vi "WaitForMessageFromAddons.vi"(8 "error in (no error)":errorcluster, 9 "timeout ms":i32=200, 10 "Name":string="Diagnostic Unlock ECU Service", 11 "TCP Ref":refnum<k5>) -> (0 "error out":errorcluster)   [LabVIEW 2024, in "Diagnostic Unlock ECU Service.lvlib"]
uses:
  Diagnostic Unlock ECU Service.lvlib
  <vilib>/NI/STM/SubVIs/MetaDataElement.ctl
  <vilib>/NI/STM/TCP/TCP Read Options.ctl
  <vilib>/NI/NI VeriStand Addon Network Comm/Shared/_Types/Comm Message.ctl
  Service Shared/UnlockECU.SendSeedToWindowsAndWaitOnKeyCmd.ctl
  Service Shared/UnlockECU.SendSeedToWindowsAndWaitOnKeyResp.ctl
  <vilib>/NI/STM/TCP/TCP Write Options.ctl
  <vilib>/NI/STM/TCP/Write Meta Data (TCP Ref).vi
  <vilib>/NI/STM/TCP/Get Connection Reference (TCP).vi
  <vilib>/NI/STM/TCP/Write Meta Data (TCP Clst).vi
  <vilib>/NI/STM/TCP/Read Message (TCP).vi
  <vilib>/NI/STM/TCP/Write Message (TCP).vi
  <vilib>/NI/STM/NI STM.lvlib
  <vilib>/Utility/SystemLogging/NI_SystemLogging.lvlib
  Service Shared/Diagnostic Unlock ECU Service Shared.lvlib
  <vilib>/NI/NI VeriStand Addon Network Comm/Shared/NI VeriStand Addon Network Comm Shared.lvlib
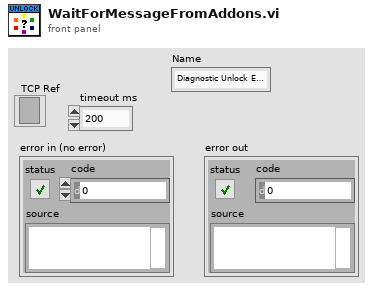
[diagram p1: front panel]
types:
  T1 = typedef "NI STM.lvlib/MetaDataElement.ctl" = string
  T2 = typedef "NI STM.lvlib/TCP Read Options.ctl" = cluster{"ignore timeout error":bool, "timeout ms (1000)":i32}
  T3 = typedef "NI VeriStand Addon Network Comm Shared.lvlib/Comm Message.ctl" = cluster{"Timeout":u32, "Resp?":bool, "data":string}
  T4 = typedef "NI STM.lvlib/TCP Write Options.ctl" = cluster{"ignore timeout error":bool, "timeout ms (1000)":i32}
  T5 = typedef "Diagnostic Unlock ECU Service Shared.lvlib/UnlockECU.SendSeedToWindowsAndWaitOnKeyResp.ctl" = cluster{"DLL Error":errorcluster, "Key Length":u32, "Key":u8[]}
  T6 = typedef "Diagnostic Unlock ECU Service Shared.lvlib/UnlockECU.SendSeedToWindowsAndWaitOnKeyCmd.ctl" = cluster{"Source DLL Path":path, "Security Level":u32, "Max Key Length":u32, "Seed":u8[], "ECU  Variant":i8, "Addon Name":string, "Optional Parameter":i8}
  T7 = typedef "NI STM.lvlib/TCP Connection Info.ctl" = cluster{"connection ID":refnum<k5>, "meta data":T1[]}
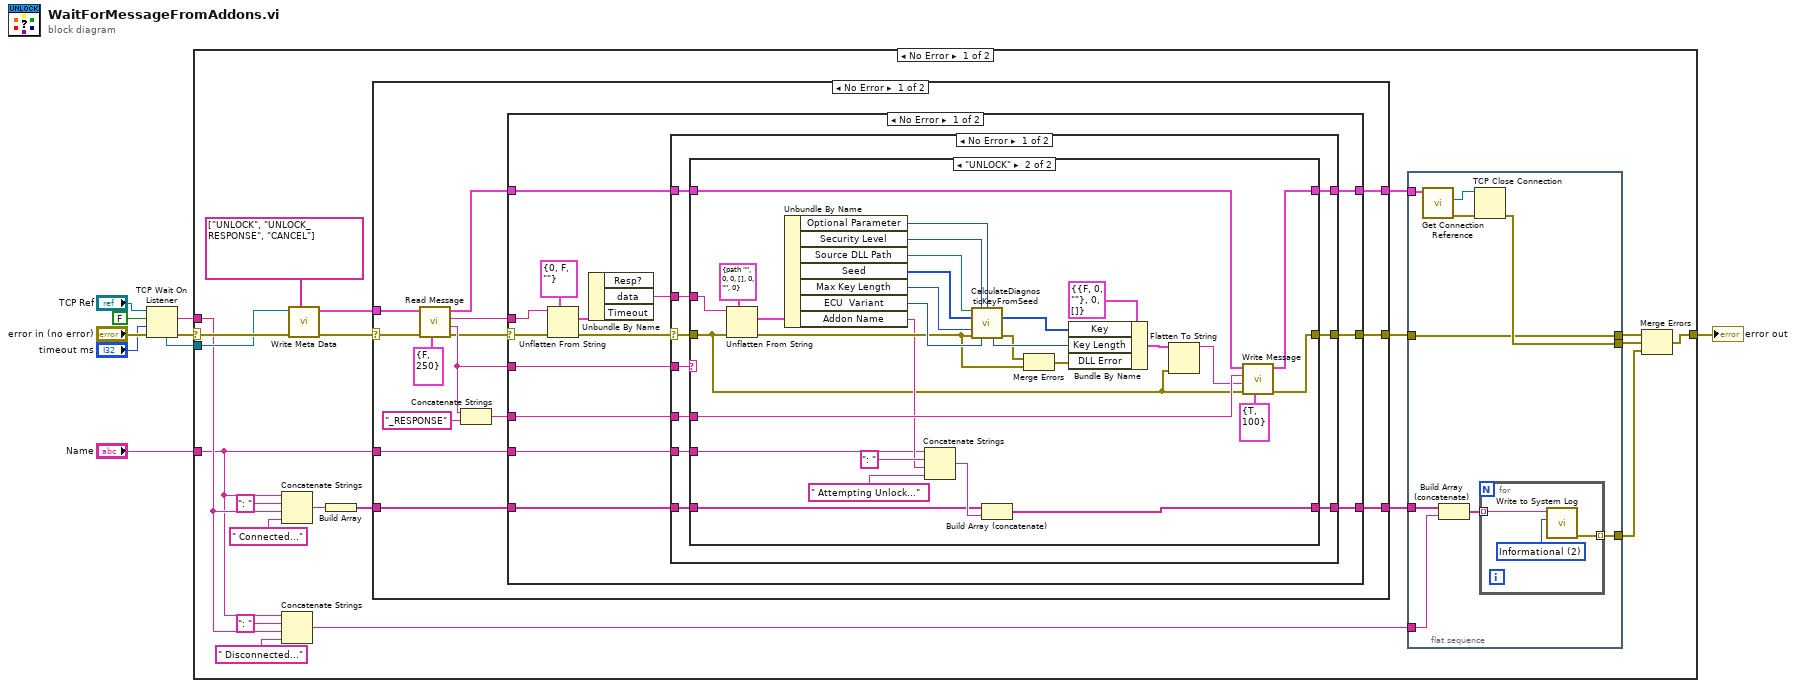
[diagram p0: block diagram]
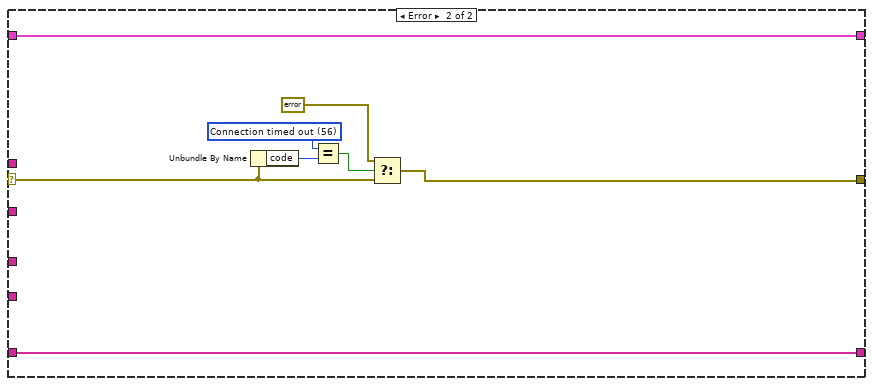
[diagram p4: hidden frame]
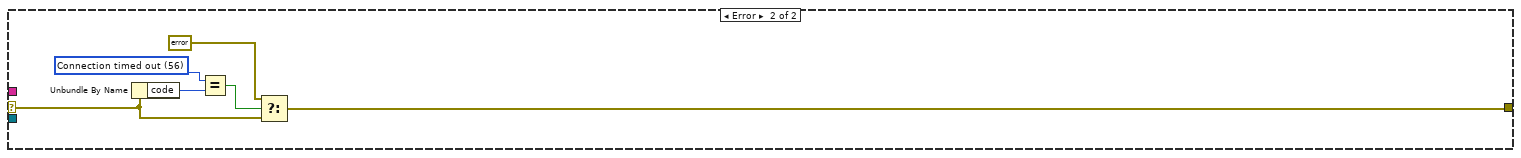
[diagram p6: hidden frame]
diagram:
  n1 = TCP Wait On Listener(8:"error in (no error)", 9:"timeout ms", 10:FALSE ("resolve remote address (T)"), 11:"TCP Ref") -> (0:w2:errorcluster, 2:w9:string, 4:w7:refnum<k5>)  [unwired: 2 out]
  n2 = case shown="No Error" w2 {
    selector: w2 -> [w30 w129]
    tunnel: [w24 w128] -> w1
    tunnel: w7 -> [w29 _]
    tunnel: w9 -> [w13 _]
    tunnel: "Name" -> [w12 _]
    frame No Error {
      n3 = Concatenate Strings(w12, ": " ("string"), w13, " Connected..." ("string")) -> (w19:string)
      n4 = Concatenate Strings(w12, ": " ("string"), w13, " Disconnected..." ("string")) -> (w11:string)
      n5 = call-poly <vilib>:"Write Meta Data.vi"("meta data"=T1[] ["UNLOCK", "UNLOCK_RESPONSE", "CANCEL"], "error in"=w30, "connection ID"=w29) -> ("error out"=w27:errorcluster, "connection info out"=w28:T7)  [unwired: 7 in]
      n6 = Build Array(w19) -> (w18:string[])
      n7 = case shown="No Error" w27 {
        selector: w27 -> [w46 w127]
        tunnel: [w48 w127] -> w22
        tunnel: w28 -> [w56 w126]
        tunnel: [w47 w126] -> w26
        tunnel: w12 -> [w45 _]
        tunnel: w18 -> [w44 w125]
        tunnel: [w43 w125] -> w17
        frame No Error {
          n8 = call-poly <vilib>:"Read Message.vi"("options"=T2 {"ignore timeout error"=FALSE, "timeout ms (1000)"=250}, "error in"=w46, "connection info in"=w56) -> ("error out"=w51:errorcluster, "name"=w53:T1, "data string"=w52:string, "connection info out"=w50:T7)  [unwired: 3 in, 2 out]
          n9 = Concatenate Strings(w53, "_RESPONSE" ("string")) -> (w49:string)
          n10 = case shown="No Error" w51 {
            selector: w51 -> [w70 w118]
            tunnel: w53 -> [w65 _]
            tunnel: w52 -> [w61 _]
            tunnel: [w69 w117] -> w48
            tunnel: w50 -> [w68 w124]
            tunnel: [w67 w124] -> w47
            tunnel: w49 -> [w66 _]
            tunnel: w45 -> [w64 _]
            tunnel: w44 -> [w63 w123]
            tunnel: [w62 w123] -> w43
            frame No Error {
              n11 = Unflatten From String(type=T3 {"Timeout"=0, "Resp?"=FALSE, "data"=""} ("Cluster"), binary string=w61, error in (no error)=w70) -> (value=w59:T3, error out=w57:errorcluster)  [unwired: 2 in, 1 out]
              n12 = Unbundle By Name(w59) -> ("data"=w58:string)  [unwired: 2 out]
              n13 = case shown="No Error" w57 {
                selector: w57 -> [w71 w116]
                tunnel: [w80 w116] -> w69
                tunnel: w68 -> [w79 w115]
                tunnel: [w78 w115] -> w67
                tunnel: w66 -> [w77 _]
                tunnel: w65 -> [w76 _]
                tunnel: w64 -> [w75 _]
                tunnel: w63 -> [w74 w114]
                tunnel: [w73 w114] -> w62
                tunnel: w58 -> [w72 _]
                frame No Error {
                  n14 = case shown="\"UNLOCK\"" w76 {
                    tunnel: w71 -> [w83 w85]
                    tunnel: [w83 w90] -> w80
                    tunnel: w79 -> [w82 w111]
                    tunnel: [w82 w110] -> w78
                    tunnel: w77 -> [_ w109]
                    tunnel: w75 -> [_ w91]
                    tunnel: w74 -> [w81 w88]
                    tunnel: [w81 w87] -> w73
                    tunnel: w72 -> [_ w84]
                    frame "CANCEL", Default {
                    }
                    frame "UNLOCK" {
                      n15 = Unflatten From String(type=T6 {"Source DLL Path"=path "", "Security Level"=0, "Max Key Length"=0, "Seed"=[], "ECU  Variant"=0, "Addon Name"="", "Optional Parameter"=0} ("Settings"), binary string=w84, error in (no error)=w85) -> (value=w112:T6, error out=w97:errorcluster)  [unwired: 2 in, 1 out]
                      n16 = Unbundle By Name(w112) -> ("Optional Parameter"=w86:i8, "Security Level"=w104:u32, "Source DLL Path"=w108:path, "Seed"=w107:u8[], "Max Key Length"=w106:u32, "ECU  Variant"=w105:i8, "Addon Name"=w92:string)
                      n17 = Concatenate Strings(w91, ": " ("string"), w92, " Attempting Unlock..." ("string")) -> (w89:string)
                      n18 = call "CalculateDiagnosticKeyFromSeed.vi"("SeedKey DLL path"=w108, "security level"=w104, "optional parameter (OEM specific)"=w86, "seed"=w107, "maximum key length"=w106, "error in (no error)"=w97, "ECU variant"=w105) -> ("key"=w102:u8[], "key length"=w101:u32, "error out"=w96:errorcluster)  [unwired: 5 in, 1 out]
                      n19 = Build Array (concatenate)(w88, w89) -> (w87:string[])
                      n20 = Merge Errors(w96, w97) -> (w95:errorcluster)
                      n21 = Bundle By Name(cluster=T5 {"DLL Error"={"status"=FALSE, "code"=0, "source"=""}, "Key Length"=0, "Key"=[]} ("Cluster"), "Key"=w102, "Key Length"=w101, "DLL Error"=w95) -> (w100:T5)
                      n22 = Flatten To String(anything=w100, error in (no error)=w85) -> (data string=w99:string)  [unwired: 2 in, 2 out]
                      n23 = call-poly <vilib>:"Write Message.vi"("options"=T4 {"ignore timeout error"=TRUE, "timeout ms (1000)"=100}, "error in"=w85, "data"=w99, "name"=w109, "connection info in"=w111) -> ("error out"=w90:errorcluster, "connection info out"=w110:T7)  [unwired: 5 in]
                    }
                  }
                }
                frame Error {
                }
              }
            }
            frame Error {
              w119 = 56 items=["No Error", "Argument Error", "Memory Full", "Out of Zone", "End of File", "File Already Open", "Generic File IO Error", "File Not Found", "File Permission Error", "Disk Full", "Duplicate Path", "Too Many Files Open", "Not Enabled", "Resource File Not Found", "Cannot Add Resource", "Resource Not Found", "Image Not Found", "Image Memory Error", "Pen Does Not Exist", "Config Bad Type", "Config Token Not Found", "Config Parse Error", "Config Memory Error", "Bad External Code Format", "Bad External Code Offset", "External Code Not Present", "Null Window", "Destroy Window Mixup", "Null Menu", "Print Aborted", "Bad Print Record", "Print Driver Error", "Windows Error During Print", "Memory Error During Print", "Print Dialog Error", "Generic Print Error", "Invalid Device Refnum", "Device Not Found", "Device Parameter Error", "Device Unit Error", "Can't Open Device", "Device Call Aborted", "Generic Error", "Cancelled By User", "Object ID Too Low", "Object ID Too High", "Object Not In Heap", "Unknown Heap", "Bad DefProc ID", "DefProc Not In Table", "Message Out Of Range", "Null Method", "Unknown Message", "Manager Call Not Supported", "Bad address", "Connection In progress", "Connection timed out", "Connection is already in progress", "Network attribute not supported", "Network error", "Address in use", "System out of memory", "Connection aborted", "Connection refused", "Connection is not connected", "Connection is already connected", "Connection closed", "Initialize error (interapplication manager)", "Bad occurrence", "Wait on unbound occurrence handler", "Occurrence queue overflow", "Bad path", "Semaphore not signaled", "Unrecognized type (interapplication manager)"] ("1st Error to Convert")
              n24 = Unbundle By Name(w118) -> ("code"=w121:i32)
              n25 = Equal?(x=w119, y=w121) -> (x = y?=w122:bool)
              n26 = Select(t=errorcluster {"status"=FALSE, "code"=0, "source"=""} ("error in (no error)"), s=w122, f=w118) -> (s? t:f=w117:errorcluster)
            }
          }
        }
        frame Error {
        }
      }
      n27 = flat-sequence {
        tunnel: w26 -> [w38]
        tunnel: [w36] -> w25
        tunnel: [w35] -> w16
        tunnel: [w34] -> w23
        tunnel: w22 -> [w34]
        tunnel: w17 -> [w33]
        tunnel: w11 -> [w31]
        frame #0 {
          n28 = call-poly <vilib>:"Get Connection Reference.vi"("connection info in"=w38) -> ("error out"=w37:errorcluster, "connection ID out"=w39:refnum<k5>)  [unwired: 8 in, 1 out]
          n29 = Build Array (concatenate)(w33, w31) -> (w32:string[])
          n30 = TCP Close Connection(connection ID=w39, error in (no error)=w37) -> (error out=w36:errorcluster)  [unwired: 1 in, 1 out]
          n31 = for {
            tunnel: w32 -> [w41] mode=indexing
            tunnel: [w40] -> w35 mode=indexing
            w42 = 2 items=["Error", "Warning", "Informational"] ("severity")
            n32 = call <vilib>:"Write to System Log.vi"("severity"=w42, "message"=w41) -> ("error out"=w40:errorcluster)  [unwired: 9 in]
          }
        }
      }
      n33 = Merge Errors(w23, w25, w16) -> (w24:errorcluster)
    }
    frame Error {
      w130 = 56 items=["No Error", "Argument Error", "Memory Full", "Out of Zone", "End of File", "File Already Open", "Generic File IO Error", "File Not Found", "File Permission Error", "Disk Full", "Duplicate Path", "Too Many Files Open", "Not Enabled", "Resource File Not Found", "Cannot Add Resource", "Resource Not Found", "Image Not Found", "Image Memory Error", "Pen Does Not Exist", "Config Bad Type", "Config Token Not Found", "Config Parse Error", "Config Memory Error", "Bad External Code Format", "Bad External Code Offset", "External Code Not Present", "Null Window", "Destroy Window Mixup", "Null Menu", "Print Aborted", "Bad Print Record", "Print Driver Error", "Windows Error During Print", "Memory Error During Print", "Print Dialog Error", "Generic Print Error", "Invalid Device Refnum", "Device Not Found", "Device Parameter Error", "Device Unit Error", "Can't Open Device", "Device Call Aborted", "Generic Error", "Cancelled By User", "Object ID Too Low", "Object ID Too High", "Object Not In Heap", "Unknown Heap", "Bad DefProc ID", "DefProc Not In Table", "Message Out Of Range", "Null Method", "Unknown Message", "Manager Call Not Supported", "Bad address", "Connection In progress", "Connection timed out", "Connection is already in progress", "Network attribute not supported", "Network error", "Address in use", "System out of memory", "Connection aborted", "Connection refused", "Connection is not connected", "Connection is already connected", "Connection closed", "Initialize error (interapplication manager)", "Bad occurrence", "Wait on unbound occurrence handler", "Occurrence queue overflow", "Bad path", "Semaphore not signaled", "Unrecognized type (interapplication manager)"] ("1st Error to Convert")
      n34 = Unbundle By Name(w129) -> ("code"=w132:i32)
      n35 = Equal?(x=w130, y=w132) -> (x = y?=w133:bool)
      n36 = Select(t=errorcluster {"status"=FALSE, "code"=0, "source"=""} ("error in (no error)"), s=w133, f=w129) -> (s? t:f=w128:errorcluster)
    }
  }
  "error out" <- w1
